vi "Listen To Msg.vi"(7 "Actor in":refnum<class "Actor.lvclass">, 10 "Msg":refnum<class "Msg.lvclass">) -> (0 "Error out":errorcluster, 2 "Msg Output":refnum<class "Msg Output.lvclass">, 5 "Actor out":refnum<class "Actor.lvclass">)   [LabVIEW 2020, in "jettl.lvlib"]
uses:
  jettl.lvlib
  Actor/Actor.lvclass
  Msg/Msg.lvclass
  Msg Output/Msg Output.lvclass
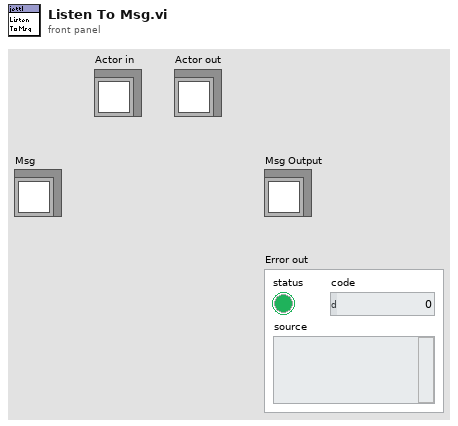
[diagram p1: front panel]
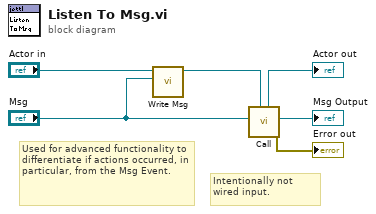
[diagram p0: block diagram]
diagram:
  # "Intentionally not wired input."
  # "Used for advanced functionality to differentiate if actions occurred, in particular, from the Msg Event."
  n1 = call-dynamic "Write Msg.vi"("Msg"="Msg", "Actor in"="Actor in") -> ("Actor out"=w3:refnum<class "Actor.lvclass">)  [unwired: 9 in]
  n2 = call "Call.vi"("Actor in"=w3, "Msg"="Msg") -> ("Error out"=→"Error out":errorcluster, "Msg Output"=→"Msg Output":refnum<class "Msg Output.lvclass">, "Actor out"=→"Actor out":refnum<class "Actor.lvclass">)  [unwired: 7 in]
